vi "Get X and Y (multiple).vi"(8 "error in (no error)":errorcluster, 11 "XY-data":cluster{"X-array":dbl[], "Y-array":dbl[]}[](array[cluster]) {"Y-array" format="%.2p"; "X-array" format="%.2p"}) -> (0 "error out":errorcluster, 1 "Y-Arrays":cluster{"Y-array":dbl[]}[](array[cluster]), 2 "X-Arrays":cluster{"X-array":dbl[]}[](array[cluster]), 3 "XY-data out":cluster{"X-array":dbl[], "Y-array":dbl[]}[](array[cluster]) {"Y-array" format="%.2p"; "X-array" format="%.2p"})   [LabVIEW 2019, in "xy_utilities.lvlib"]
doc: "Returns the X and Y arrays contained in <b>XY-data</b>.\n\nWire data to the data input to determine the polymorphic instance to use or manually select the instance."
uses:
  xy_utilities.lvlib
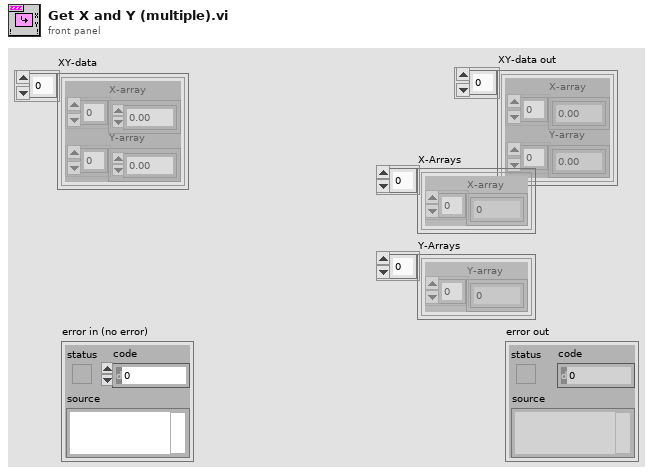
[diagram p1: front panel]
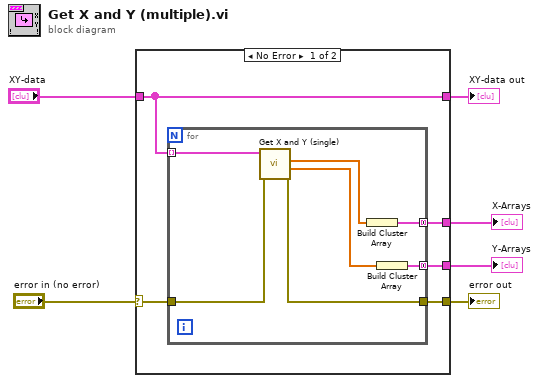
[diagram p0: block diagram]
diagram:
  n1 = case shown="No Error" "error in (no error)" {
    selector: "error in (no error)" -> [w11 w20]
    tunnel: [w10 w20] -> w5
    tunnel: "XY-data" -> [w7 w19]
    tunnel: [w7 w19] -> w3
    tunnel: [w9 _] -> w2
    tunnel: [w8 _] -> w1
    frame No Error {
      n2 = for {
        tunnel: w7 -> [w18] mode=indexing
        tunnel: [w14] -> w9 mode=concatenating
        tunnel: [w15] -> w8 mode=concatenating
        tunnel: w11 -> [w13]
        tunnel: [w12] -> w10
        n3 = call "Get X and Y (single).vi"("error in (no error)"=w13, "XY-data"=w18) -> ("error out"=w12:errorcluster, "Y-array"=w16:dbl[], "X-array"=w17:dbl[])  [unwired: 6 in, 1 out]
        n4 = Build Cluster Array(w17) -> (w14:cluster{"X-array":dbl[]}[])
        n5 = Build Cluster Array(w16) -> (w15:cluster{"Y-array":dbl[]}[])
      }
    }
    frame Error {
    }
  }
  "error out" <- w5
  "XY-data out" <- w3
  "X-Arrays" <- w2
  "Y-Arrays" <- w1
